vi "Add Custom Device Channel - Offline.vi"(4 "Property Values":variant[](array[variant]), 5 "Highlight? (F)":bool, 6 "Property names":string[](array[string]), 7 "GUID (Default Channel)":string="03D3BB99-1485-13A6-561D1F898F032919", 8 "error in (no error)":errorcluster, 9 "Channel":T2, 10 "Channel Name":string, 11 "Parent Ref in":T1 format="%.0x") -> (0 "error out":errorcluster, 1 "Channel Ref":T1 format="%.0x", 2 "Newly Created?":bool, 3 "Parent Ref out":T1 format="%.0x")   [LabVIEW 2027, in "SEECD System Explorer.lvlib"]
uses:
  SEECD System Explorer.lvlib
  <vilib>/NI VeriStand/Custom Device Offline API/Custom Device Offline API.lvlib
  <vilib>/NI VeriStand/Custom Device API/Custom Device Item Ref.ctl
  <vilib>/NI VeriStand/Custom Device API/Custom Device API.lvlib
  C:/NetCoreDLL/NationalInstruments.VeriStand.SystemDefinitionAPI.dll
  NetCoreDLL/NationalInstruments.VeriStand.SystemDefinitionAPI.dll
  <vilib>/NI VeriStand/Custom Device API/Custom Device Channel Type.ctl
  <vilib>/NI VeriStand/Custom Device API/Custom Device Channel.ctl
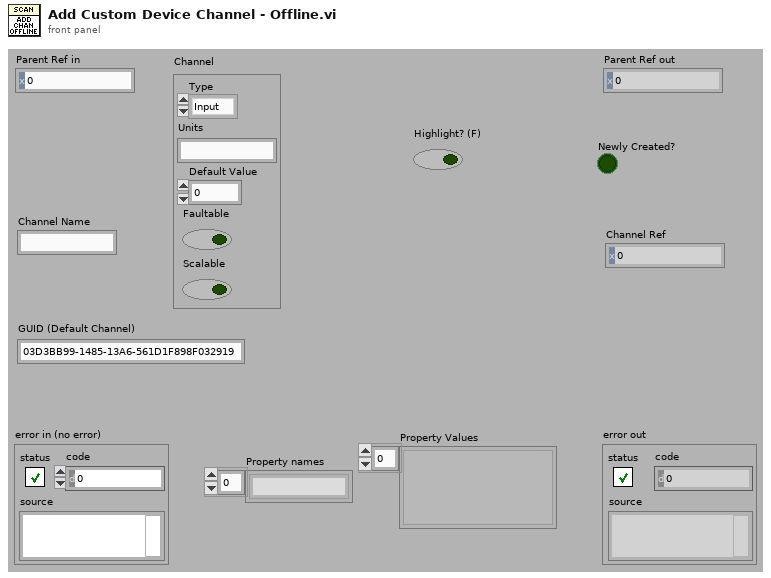
[diagram p1: front panel]
types:
  T1 = typedef "Custom Device API.lvlib/Custom Device Item Ref.ctl" = u64
  T2 = typedef "Custom Device API.lvlib/Custom Device Channel.ctl" = cluster{"Type":T3, "Units":string, "Default Value":dbl, "Faultable":bool, "Scalable":bool}
  T3 = typedef "Custom Device API.lvlib/Custom Device Channel Type.ctl" = enum16{"Input", "Output"}
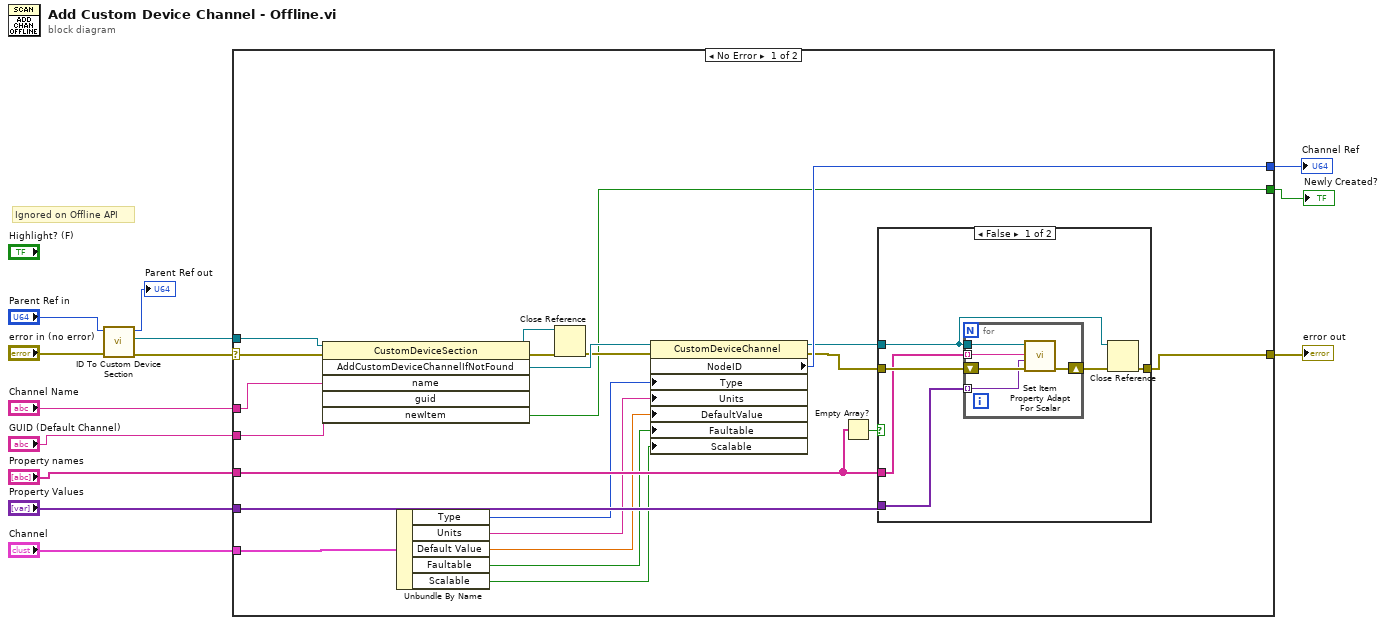
[diagram p0: block diagram]
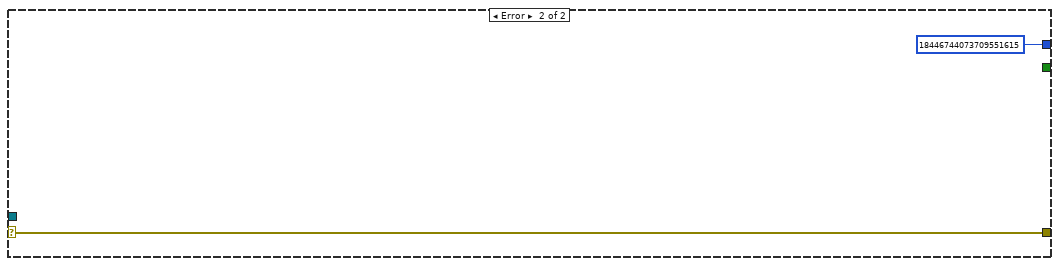
[diagram p3: hidden frame]
diagram:
  # "Ignored on Offline API"
  n1 = call <vilib>:"ID To Custom Device Section.vi"("error in (no error)"="error in (no error)", "ID in"="Parent Ref in") -> ("error out"=w13:errorcluster, "Section"=w1:refnum<k39>, "ID out"=→"Parent Ref out":u64)  [unwired: 7 in]
  n2 = case shown="No Error" w13 {
    selector: w13 -> [w35 w49]
    tunnel: [w33 w49] -> w3
    tunnel: "GUID (Default Channel)" -> [w34 _]
    tunnel: [w28 T1 18446744073709551615 ("Section Ptr")] -> w4
    tunnel: [w25 _] -> w5
    tunnel: "Property names" -> [w24 _]
    tunnel: "Property Values" -> [w23 _]
    tunnel: "Channel Name" -> [w22 _]
    tunnel: "Channel" -> [w21 _]
    tunnel: w1 -> [w14 _]
    frame No Error {
      n3 = invoke class="CustomDeviceSection" method="AddCustomDeviceChannelIfNotFound"(reference=w14, error in=w35, "name"=w22, "guid"=w34) -> (reference out=w31:refnum<k39>, error out=w32:errorcluster, "AddCustomDeviceChannelIfNotFound"=w30:refnum<k39>, "newItem"=w25:bool)  [unwired: 2 in, 2 out]
      n4 = Unbundle By Name(w21) -> ("Type"=w20:T3, "Units"=w19:string, "Default Value"=w18:dbl, "Faultable"=w17:bool, "Scalable"=w16:bool)
      n5 = Close Reference(reference=w31, error in (no error)=w32) -> (error out=w29:errorcluster)
      n6 = property class="CustomDeviceChannel"(reference=w30, error in=w29, "Type"=w20, "Units"=w19, "DefaultValue"=w18, "Faultable"=w17, "Scalable"=w16) -> (reference out=w26:refnum<k39>, error out=w27:errorcluster, "NodeID"=w28:u64)
      n7 = Empty Array?(array=w24) -> (empty?=w15:bool)
      n8 = case shown="False" w15 {
        tunnel: w26 -> [w37 _]
        tunnel: w27 -> [w41 w47]
        tunnel: w23 -> [w40 _]
        tunnel: w24 -> [w39 _]
        tunnel: [w36 w47] -> w33
        frame False {
          n9 = for {
            tunnel: w40 -> [w45] mode=indexing
            tunnel: w39 -> [w44] mode=indexing
            shift-right: [w42] -> w38
            shift-left: w41 -> [w46]
            tunnel: w37 -> [w43]
            n10 = call <vilib>:"Set Item Property Adapt For Scalar.vi"("error in (no error)"=w46, "Value"=w45, "Property Name"=w44, "NationalInstruments.VeriStand.SystemDefinitionAPI.CustomDeviceBase"=w43) -> ("error out"=w42:errorcluster)  [unwired: 5 in, 2 out]
          }
          n11 = Close Reference(reference=w37, error in (no error)=w38) -> (error out=w36:errorcluster)
        }
        frame True {
        }
      }
    }
    frame Error {
    }
  }
  "error out" <- w3
  "Channel Ref" <- w4
  "Newly Created?" <- w5
